vi "Create Boolean Channel.vi"(7 "Input?":bool, 8 "error in (no error)":errorcluster, 10 "Channel Number":i32) -> (0 "error out":errorcluster, 2 "Boolean Channel":T1, 3 "Channel out":refnum<class "Channel.lvclass">)   [LabVIEW 2026, in "Modbus.lvlib" / "Modbus.lvclass"]
uses:
  Modbus.lvclass
  <vilib>/FlexLogger/SDK/PluginSDK.lvlibp/PEFClasses/SDK/Channel/Channel.lvclass
  Types/Boolean Data.ctl
  Types/Modbus Table.ctl
  <vilib>/FlexLogger/SDK/PluginSDK.lvlibp/PEFClasses/SDK/Channel/Data Type.ctl
  <vilib>/FlexLogger/SDK/PluginSDK.lvlibp/PEFClasses/SDK/Channel/Data Type_v2.ctl
  e0cdf0dc-ec87-4ce3-9d59-fa7e6132dbb7.vi
  <vilib>/FlexLogger/SDK/PluginSDK.lvlibp/PEFClasses/SDK/Setpoint Consumer Channel/Setpoint Consumer Channel.lvclass
  <vilib>/FlexLogger/SDK/PluginSDK.lvlibp/PEFClasses/SDK/Producer Channel/Producer Channel.lvclass
  Globals/Modbus Strings.vi
  <vilib>/FlexLogger/SDK/PluginSDK.lvlibp/PEFClasses/SDK/Setpoint Consumer Channel/Create Setpoint Consumer Channel_v2.vi
  <vilib>/FlexLogger/SDK/PluginSDK.lvlibp/PEFClasses/SDK/Producer Channel/Create Producer Channel_v2.vi
  <vilib>/FlexLogger/SDK/PluginSDK.lvlibp/PEFClasses/SDK/Channel/ParameterAccess/Write Enum.vi
  <vilib>/FlexLogger/SDK/PluginSDK.lvlibp/PEFClasses/SDK/Channel/ParameterAccess/Write I32.vi
  <vilib>/FlexLogger/SDK/PluginSDK.lvlibp
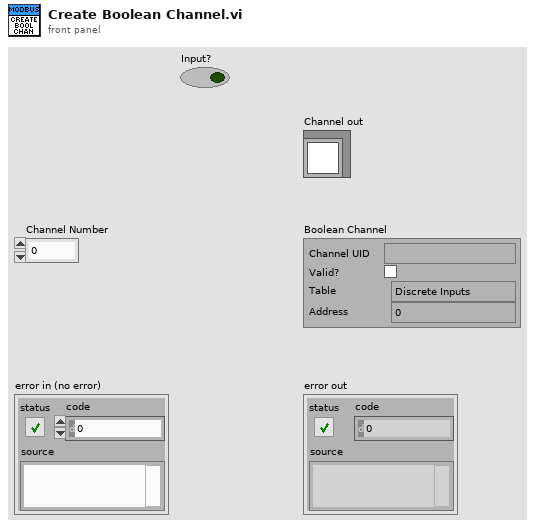
[diagram p1: front panel]
types:
  T1 = typedef "Modbus.lvlib/Modbus.lvclass/Boolean Data.ctl" = cluster{"Channel UID":string, "Valid?":bool, "Table":T2, "Address":i32}
  T2 = typedef "Modbus.lvlib/Modbus.lvclass/Modbus Table.ctl" = enum16{"Discrete Inputs", "Coils", "Input Registers", "Holding Registers"}
  T3 = typedef "PluginSDK.lvlibp/Channel.lvclass/Data Type.ctl" = enum16{"Wfm (DBL)", "Wfm (Digital)"}
  T4 = typedef "PluginSDK.lvlibp/Channel.lvclass/Data Type_v2.ctl" = u16
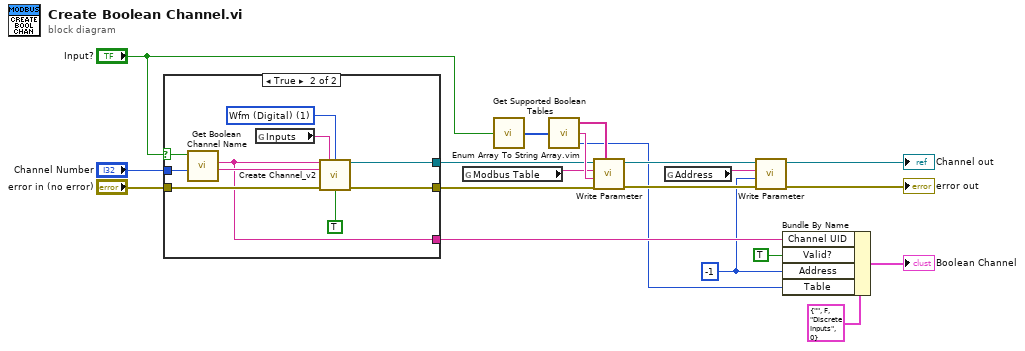
[diagram p0: block diagram]
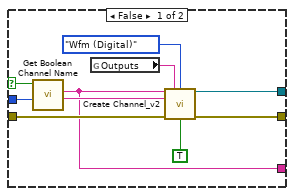
[diagram p2: hidden frame]
diagram:
  w2 = -1 ("Value")
  n1 = case shown="True" "Input?" {
    selector: "Input?" -> [w24 w35]
    tunnel: "error in (no error)" -> [w27 w37]
    tunnel: [w29 w39] -> w10
    tunnel: [w30 w40] -> w11
    tunnel: "Channel Number" -> [w21 w32]
    tunnel: [w22 w33] -> w20
    frame False {
      n2 = call "Get Boolean Channel Name.vi"("Channel Numer"=w21, "Input?"=w24) -> ("Bool Channel Name"=w23:string, "Bool Channel ID"=w22:string)  [unwired: 8 in]
      n3 = global read "Modbus Strings.vi" "Outputs"() -> (w28:string)
      n4 = call-poly <vilib>:"Create Channel_v2.vi"("Unique Channel Identifier"=w22, "Display Group"=w28, "Data Type"=Data_Type."Wfm (Digital)", "Default Channel Name"=w23, "error in (no error)"=w27, "Can Disable?"=TRUE) -> ("Setpoint Consumer Channel"=w29:refnum<class "Setpoint Consumer Channel.lvclass">, "error out"=w30:errorcluster)  [unwired: 8 in]
    }
    frame True {
      w31 = T4 1 items=["Wfm (DBL)", "Wfm (Digital)", "String"] ("Data Type")
      n5 = call "Get Boolean Channel Name.vi"("Channel Numer"=w32, "Input?"=w35) -> ("Bool Channel Name"=w34:string, "Bool Channel ID"=w33:string)  [unwired: 8 in]
      n6 = global read "Modbus Strings.vi" "Inputs"() -> (w38:string)
      n7 = call-poly <vilib>:"Create Channel_v2.vi"("Unique Channel Identifier"=w33, "Display Group"=w38, "Data Type"=w31, "Default Channel Name"=w34, "error in (no error)"=w37, "Can Disable?"=TRUE) -> ("Producer Channel"=w39:refnum<class "Producer Channel.lvclass">, "error out"=w40:errorcluster)  [unwired: 8 in]
    }
  }
  n8 = global read "Modbus Strings.vi" "Modbus Table"() -> (w8:string)
  n9 = call "Get Supported Boolean Tables.vi"("Input?"="Input?") -> ("Supported Tables"=w19:T2[])
  n10 = call "Enum Array To String Array.vim"("Array of Enum Values"=w19) -> ("First Value"=w3:T2, "First String"=w13:string, "Strings out"=w12:string[])  [unwired: 2 in]
  n11 = call-poly <vilib>:"Write Parameter.vi"("Possible Values"=w12, "error in (no error)"=w11, "Current Value"=w13, "Name"=w8, "Channel in"=w10) -> ("error out"=w5:errorcluster, "Channel out"=w4:refnum<class "Channel.lvclass">)  [unwired: 5 in]
  n12 = global read "Modbus Strings.vi" "Address"() -> (w9:string)
  n13 = call-poly <vilib>:"Write Parameter.vi"("error in (no error)"=w5, "Value"=w2, "Name"=w9, "Channel in"=w4) -> ("error out"=→"error out":errorcluster, "Channel out"=→"Channel out":refnum<class "Channel.lvclass">)  [unwired: 6 in]
  n14 = Bundle By Name(cluster=T1 {"Channel UID"="", "Valid?"=FALSE, "Table"=enum."Discrete Inputs", "Address"=0} ("Boolean Data"), "Channel UID"=w20, "Valid?"=TRUE, "Address"=w2, "Table"=w3) -> (→"Boolean Channel":T1)
